vi "Decode Schedule Message.vi"(8 "error in (no error)":errorcluster, 10 "Schedules":refnum<class "Schedule.lvclass">[](array[class]), 11 "Tamer in":refnum<class "Tamer.lvclass">) -> (0 "error out":errorcluster, 3 "Tamer out":refnum<class "Tamer.lvclass">)   [LabVIEW 2020, in "Tamer.lvlib" / "Tamer.lvclass"]
uses:
  Tamer.lvclass
  Tamer.lvclass/Tamer.ctl
  Run Utilities/TypeDefs/Monkey Status.ctl
  Run Utilities/Schedule/Schedule.lvclass
  Run Utilities/Run Utilities.lvlib
  Run Utilities/TypeDefs/Synchronize FPGA Cluster.ctl
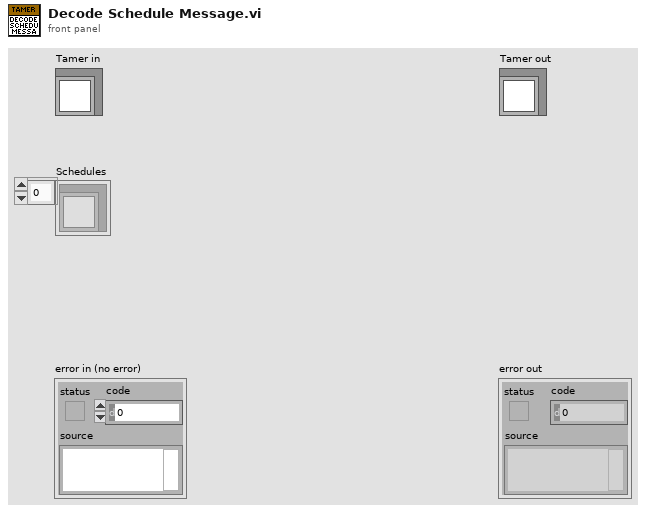
[diagram p1: front panel]
types:
  T1 = typedef "Run Utilities.lvlib/Monkey Status.ctl" = enum16{"Init", "Paused", "Ongoing", "Stopped", "Finished (no errors)", "Finished (with errors)"}
  T2 = typedef "Run Utilities.lvlib/Synchronize FPGA Cluster.ctl" = cluster{"Status":bool, "FPGA Name":string}
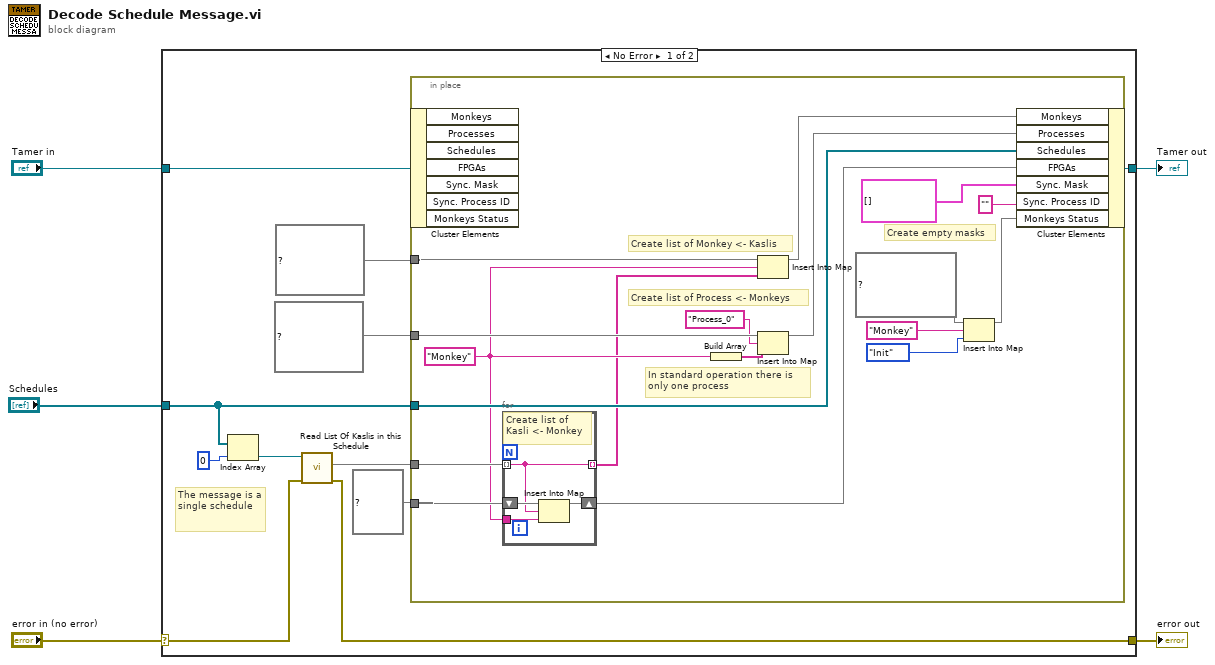
[diagram p0: block diagram]
diagram:
  n1 = case shown="No Error" "error in (no error)" {
    selector: "error in (no error)" -> [w14 w40]
    tunnel: [w7 w40] -> w4
    tunnel: [w8 w39] -> w2
    tunnel: "Tamer in" -> [w11 w39]
    tunnel: "Schedules" -> [w6 _]
    frame No Error {
      # "The message is a single schedule"
      n2 = Index Array(array=w6, index=0) -> (element=w15:refnum<class "Schedule.lvclass">)
      n3 = call-dynamic "Read List Of Kaslis in this Schedule.vi"("error in (no error)"=w14, "Schedule in"=w15) -> ("error out"=w7:errorcluster, "List of FPGAs"=w13:set{string})  [unwired: 7 in, 1 out]
      n4 = in-place {
        in-place-border: w13 -> [w31]
        in-place-border: map{string, string[]} {} ("Monkeys") -> [w34]
        in-place-border: w6 -> [w29]
        in-place-border: map{string, string} {} ("Kaslis") -> [w32]
        in-place-border: map{string, string[]} {} ("Processes") -> [w28]
        w24 = "Monkey" ("key")
        # "Create empty masks"
        # "In standard operation there is only one process"
        # "Create list of Process <- Monkeys"
        # "Create list of Monkey <- Kaslis"
        n5 = in-place-cluster #1(w11) -> ()  [unwired: 7 out]
        n6 = for {
          tunnel: w31 -> [w35] mode=indexing
          shift-right: [w37] -> w30
          shift-left: w32 -> [w38]
          tunnel: w24 -> [w36]
          tunnel: [w35] -> w17 mode=indexing
          # "Create list of Kasli <- Monkey"
          n7 = Insert Into Map(map in=w38, key=w35, value=w36) -> (map out=w37:map{string, string})  [unwired: 2 out]
        }
        n8 = Build Array(w24) -> (w25:string[])
        n9 = Insert Into Map(map in=w34, key=w24, value=w17) -> (map out=w33:map{string, string[]})  [unwired: 2 out]
        n10 = Insert Into Map(map in=w28, key="Process_0", value=w25) -> (map out=w26:map{string, string[]})  [unwired: 2 out]
        n11 = Insert Into Map(map in=map{string, T1} {} ("Monkeys Status"), key="Monkey", value=Monkey_Status."Init") -> (map out=w21:map{string, T1})  [unwired: 2 out]
        n12 = in-place-cluster #1("Monkeys"=w33, "Processes"=w26, "Schedules"=w29, "FPGAs"=w30, "Sync. Mask"=T2[] [] ("Synchronize Mask"), "Sync. Process ID"="" ("Parallel Process ID"), "Monkeys Status"=w21) -> (w8:refnum<class "Tamer.lvclass">)
      }
    }
    frame Error {
    }
  }
  "error out" <- w4
  "Tamer out" <- w2
